vi "T2_Tau_Manipulation.vi"(8 "Numeric 2":i32, 9 "Invert?":bool, 10 "Numeric":i32, 11 "MW Step Size":dbl=2e-09) -> (3 "Tau":dbl)   [LabVIEW 2024]
uses:
  <vilib>/Utility/error.llb/DialogTypeEnum.ctl
  SpinCore_API_file_location.vi
panel:
  out "output array 2":T1(array[cluster])
  in  "clock_freq (MHz) 2":dbl=500.0
  out "x+y 11":dbl
  out "x+y 10":dbl
  out "x+y 9":dbl
  out "x+y 8":dbl
  out "x+y 7":dbl
  out "x+y 6":dbl
  out "x+y 5":dbl
  out "x+y 4":dbl
  out "x+y 3":dbl
  out "x+y 2":dbl
  out "output array":T1(array[cluster])
  in  "Instructions":T1(array[cluster])=[{"Instruct Data"=0, "Op Code"=0, "Flags"=[FALSE, FALSE, TRUE, FALSE, FALSE, FALSE, FALSE, TRUE, FALSE, FALSE, FALSE, FALSE, FALSE, FALSE, FALSE, FALSE, FALSE, FALSE, FALSE, FALSE, FALSE, FALSE, FALSE, TRUE], "Comments"="0 Triggers", "Time (s)"=1e-07}, {"Instruct Data"=0, "Op Code"=0, "Flags"=[FALSE, FALSE, FALSE, FALSE, FALSE, FALSE, FALSE, TRUE, FALSE, FALSE, FALSE, FALSE, FALSE, FALSE, FALSE, FALSE, FALSE, FALSE, FALSE, FALSE, FALSE, FALSE, FALSE, FALSE], "Comments"="1 Dark ", "Time (s)"=0.00017}, {"Instruct Data"=0, "Op Code"=0, "Flags"=[FALSE, FALSE, FALSE, FALSE, FALSE, FALSE, FALSE, TRUE, FALSE, FALSE, FALSE, FALSE, FALSE, FALSE, FALSE, FALSE, FALSE, FALSE, FALSE, FALSE, FALSE, FALSE, FALSE, FALSE], "Comments"="2 AOM Buffer", "Time (s)"=5e-07}, {"Instruct Data"=0, "Op Code"=0, "Flags"=[TRUE, FALSE, FALSE, TRUE, FALSE, FALSE, FALSE, TRUE, FALSE, FALSE, FALSE, FALSE, FALSE, FALSE, FALSE, FALSE, FALSE, FALSE, FALSE, FALSE, FALSE, FALSE, FALSE, FALSE], "Comments"="3 pi/2", "Time (s)"=3.7e-08}, {"Instruct Data"=0, "Op Code"=0, "Flags"=[FALSE, FALSE, FALSE, FALSE, FALSE, FALSE, FALSE, TRUE, FALSE, FALSE, FALSE, FALSE, FALSE, FALSE, FALSE, FALSE, FALSE, FALSE, FALSE, FALSE, FALSE, FALSE, FALSE, FALSE], "Comments"="4 tau", "Time (s)"=1e-08}, {"Instruct Data"=0, "Op Code"=0, "Flags"=[TRUE, FALSE, FALSE, TRUE, FALSE, FALSE, FALSE, TRUE, FALSE, FALSE, FALSE, FALSE, FALSE, FALSE, FALSE, FALSE, FALSE, FALSE, FALSE, FALSE, FALSE, FALSE, FALSE, FALSE], "Comments"="5  Pi_X", "Time (s)"=6.7e-08}, {"Instruct Data"=0, "Op Code"=0, "Flags"=[FALSE, FALSE, FALSE, FALSE, FALSE, FALSE, FALSE, TRUE, FALSE, FALSE, FALSE, FALSE, FALSE, FALSE, FALSE, FALSE, FALSE, FALSE, FALSE, FALSE, FALSE, FALSE, FALSE, FALSE], "Comments"="6 Tau", "Time (s)"=1e-08}, {"Instruct Data"=0, "Op Code"=0, "Flags"=[TRUE, FALSE, FALSE, TRUE, FALSE, FALSE, FALSE, TRUE, FALSE, FALSE, FALSE, FALSE, FALSE, FALSE, FALSE, FALSE, FALSE, FALSE, FALSE, FALSE, FALSE, FALSE, FALSE, FALSE], "Comments"="7 Pi/2", "Time (s)"=3.7e-08}, {"Instruct Data"=0, "Op Code"=0, "Flags"=[FALSE, TRUE, FALSE, FALSE, FALSE, FALSE, FALSE, TRUE, FALSE, FALSE, FALSE, FALSE, FALSE, FALSE, FALSE, FALSE, FALSE, FALSE, FALSE, FALSE, FALSE, FALSE, FALSE, FALSE], "Comments"="8 AOM", "Time (s)"=5e-07}, {"Instruct Data"=0, "Op Code"=0, "Flags"=[FALSE, TRUE, FALSE, FALSE, FALSE, FALSE, FALSE, FALSE, FALSE, FALSE, FALSE, FALSE, FALSE, FALSE, FALSE, FALSE, FALSE, FALSE, FALSE, FALSE, FALSE, FALSE, FALSE, FALSE], "Comments"="9 AOM non inhibit window", "Time (s)"=5e-07}, {"Instruct Data"=0, "Op Code"=0, "Flags"=[FALSE, TRUE, FALSE, FALSE, FALSE, FALSE, FALSE, TRUE, FALSE, FALSE, FALSE, FALSE, FALSE, FALSE, FALSE, FALSE, FALSE, FALSE, FALSE, FALSE, FALSE, FALSE, FALSE, FALSE], "Comments"="10 AOM Repolarization", "Time (s)"=4e-06}, {"Instruct Data"=0, "Op Code"=0, "Flags"=[FALSE, FALSE, FALSE, FALSE, FALSE, FALSE, FALSE, TRUE, FALSE, FALSE, FALSE, FALSE, FALSE, FALSE, FALSE, FALSE, FALSE, FALSE, FALSE, FALSE, FALSE, FALSE, FALSE, FALSE], "Comments"="11 Dark", "Time (s)"=0.00017}, {"Instruct Data"=0, "Op Code"=0, "Flags"=[FALSE, FALSE, FALSE, FALSE, FALSE, FALSE, FALSE, TRUE, FALSE, FALSE, FALSE, FALSE, FALSE, FALSE, FALSE, FALSE, FALSE, FALSE, FALSE, FALSE, FALSE, FALSE, FALSE, FALSE], "Comments"="12 AOM Buffer", "Time (s)"=5e-07}, {"Instruct Data"=0, "Op Code"=0, "Flags"=[TRUE, FALSE, FALSE, TRUE, FALSE, FALSE, FALSE, TRUE, FALSE, FALSE, FALSE, FALSE, FALSE, FALSE, FALSE, FALSE, FALSE, FALSE, FALSE, FALSE, FALSE, FALSE, FALSE, FALSE], "Comments"="13 Pi/2", "Time (s)"=3.7e-08}, {"Instruct Data"=0, "Op Code"=0, "Flags"=[FALSE, FALSE, FALSE, FALSE, FALSE, FALSE, FALSE, TRUE, FALSE, FALSE, FALSE, FALSE, FALSE, FALSE, FALSE, FALSE, FALSE, FALSE, FALSE, FALSE, FALSE, FALSE, FALSE, FALSE], "Comments"="14 tau", "Time (s)"=1e-08}, {"Instruct Data"=0, "Op Code"=0, "Flags"=[TRUE, FALSE, FALSE, FALSE, TRUE, FALSE, FALSE, TRUE, FALSE, FALSE, FALSE, FALSE, FALSE, FALSE, FALSE, FALSE, FALSE, FALSE, FALSE, FALSE, FALSE, FALSE, FALSE, FALSE], "Comments"="15 Pi_Y", "Time (s)"=6.9e-08}, {"Instruct Data"=0, "Op Code"=0, "Flags"=[FALSE, FALSE, FALSE, FALSE, FALSE, FALSE, FALSE, TRUE, FALSE, FALSE, FALSE, FALSE, FALSE, FALSE, FALSE, FALSE, FALSE, FALSE, FALSE, FALSE, FALSE, FALSE, FALSE, FALSE], "Comments"="16 tau", "Time (s)"=1e-08}, {"Instruct Data"=0, "Op Code"=0, "Flags"=[TRUE, FALSE, FALSE, TRUE, FALSE, FALSE, FALSE, TRUE, FALSE, FALSE, FALSE, FALSE, FALSE, FALSE, FALSE, FALSE, FALSE, FALSE, FALSE, FALSE, FALSE, FALSE, FALSE, FALSE], "Comments"="17 pi/2", "Time (s)"=3.7e-08}, {"Instruct Data"=0, "Op Code"=0, "Flags"=[FALSE, TRUE, FALSE, FALSE, FALSE, FALSE, FALSE, TRUE, FALSE, FALSE, FALSE, FALSE, FALSE, FALSE, FALSE, FALSE, FALSE, FALSE, FALSE, FALSE, FALSE, FALSE, FALSE, FALSE], "Comments"="18 AOM Delay", "Time (s)"=5e-07}, {"Instruct Data"=0, "Op Code"=0, "Flags"=[FALSE, TRUE, FALSE, FALSE, FALSE, FALSE, FALSE, FALSE, FALSE, FALSE, FALSE, FALSE, FALSE, FALSE, FALSE, FALSE, FALSE, FALSE, FALSE, FALSE, FALSE, FALSE, FALSE, FALSE], "Comments"="19 AOM non inhibit window", "Time (s)"=5e-07}, {"Instruct Data"=0, "Op Code"=6, "Flags"=[FALSE, TRUE, FALSE, FALSE, FALSE, FALSE, FALSE, TRUE, FALSE, FALSE, FALSE, FALSE, FALSE, FALSE, FALSE, FALSE, FALSE, FALSE, FALSE, FALSE, FALSE, FALSE, FALSE, FALSE], "Comments"="20  AOM Repolarization", "Time (s)"=4e-06}] {"Time (s)" format="%.3p"; "Op Code" items=["Continue", "Stop", "Loop", "End Loop", "JSR", "RTS", "Branch", "Long Delay", "Wait"]}
  in  "# of Instructions":u32=21
  in  "clock_freq (MHz)":dbl=500.0
  # "1)MW indicator\n2)AOM\n3)SR400 trigger\n4) I\n5) Q\n8) Inhibit\n24) Scope Trigger"
  # "1"
  # "2"
  # "3"
  # "4"
  # "5"
  # "6"
  # "7"
  # "8"
  # "9"
  # "10"
  # "11"
  # "12"
  # "13"
  # "14"
  # "15"
  # "16"
  # "17"
  # "18"
  # "19"
  # "20"
  # "21"
  # "22"
  # "23"
  # "24"
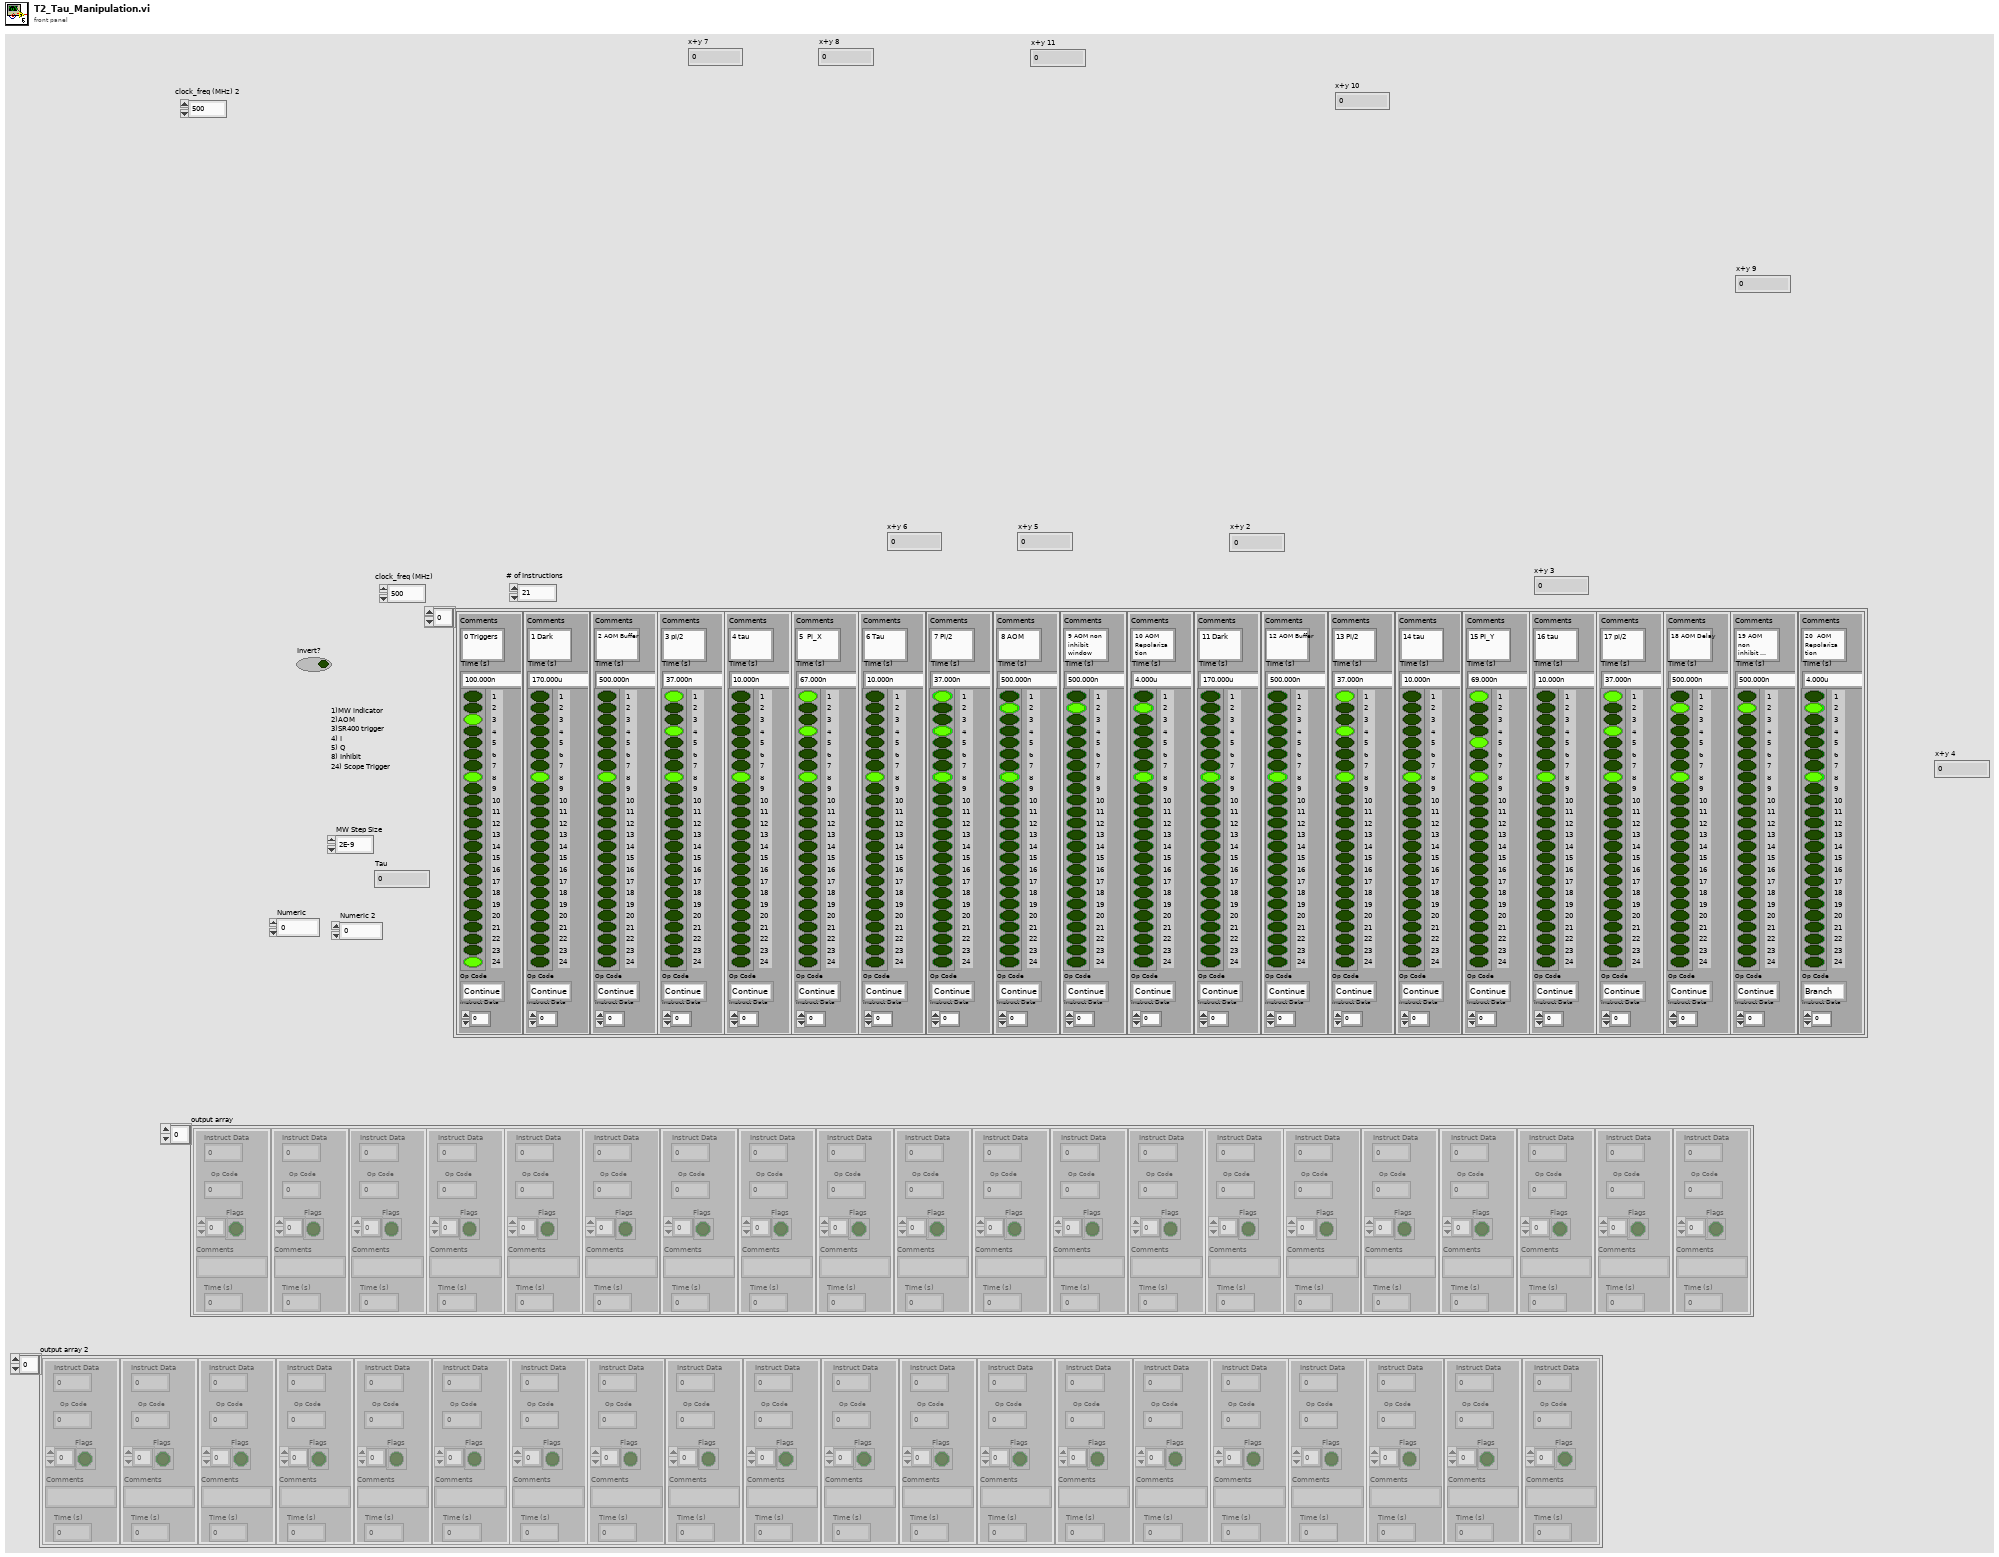
[diagram p1: front panel]
types:
  T1 = cluster{"Instruct Data":i32, "Op Code":i32, "Flags":bool[], "Comments":string, "Time (s)":dbl}[]
  T2 = typedef "DialogTypeEnum.ctl" = enum16{"no dialog", "OK message", "continue or stop message", "auto error handling dialog", "OK message + warnings", "continue/stop + warnings"}
  T3 = enum16{"Pulse Program", "Frequency Registers", "TX Phase Registers", "RX Phase Registers"}
  T4 = cluster{"Instruct Data":i32, "Op Code":i32, "Flags":bool[], "Comments":string, "Time (s)":dbl}
  T5 = cluster{"Instruct Data":i32, "Op Code":i32, "Flags":bool[], "Comments":string, dbl}
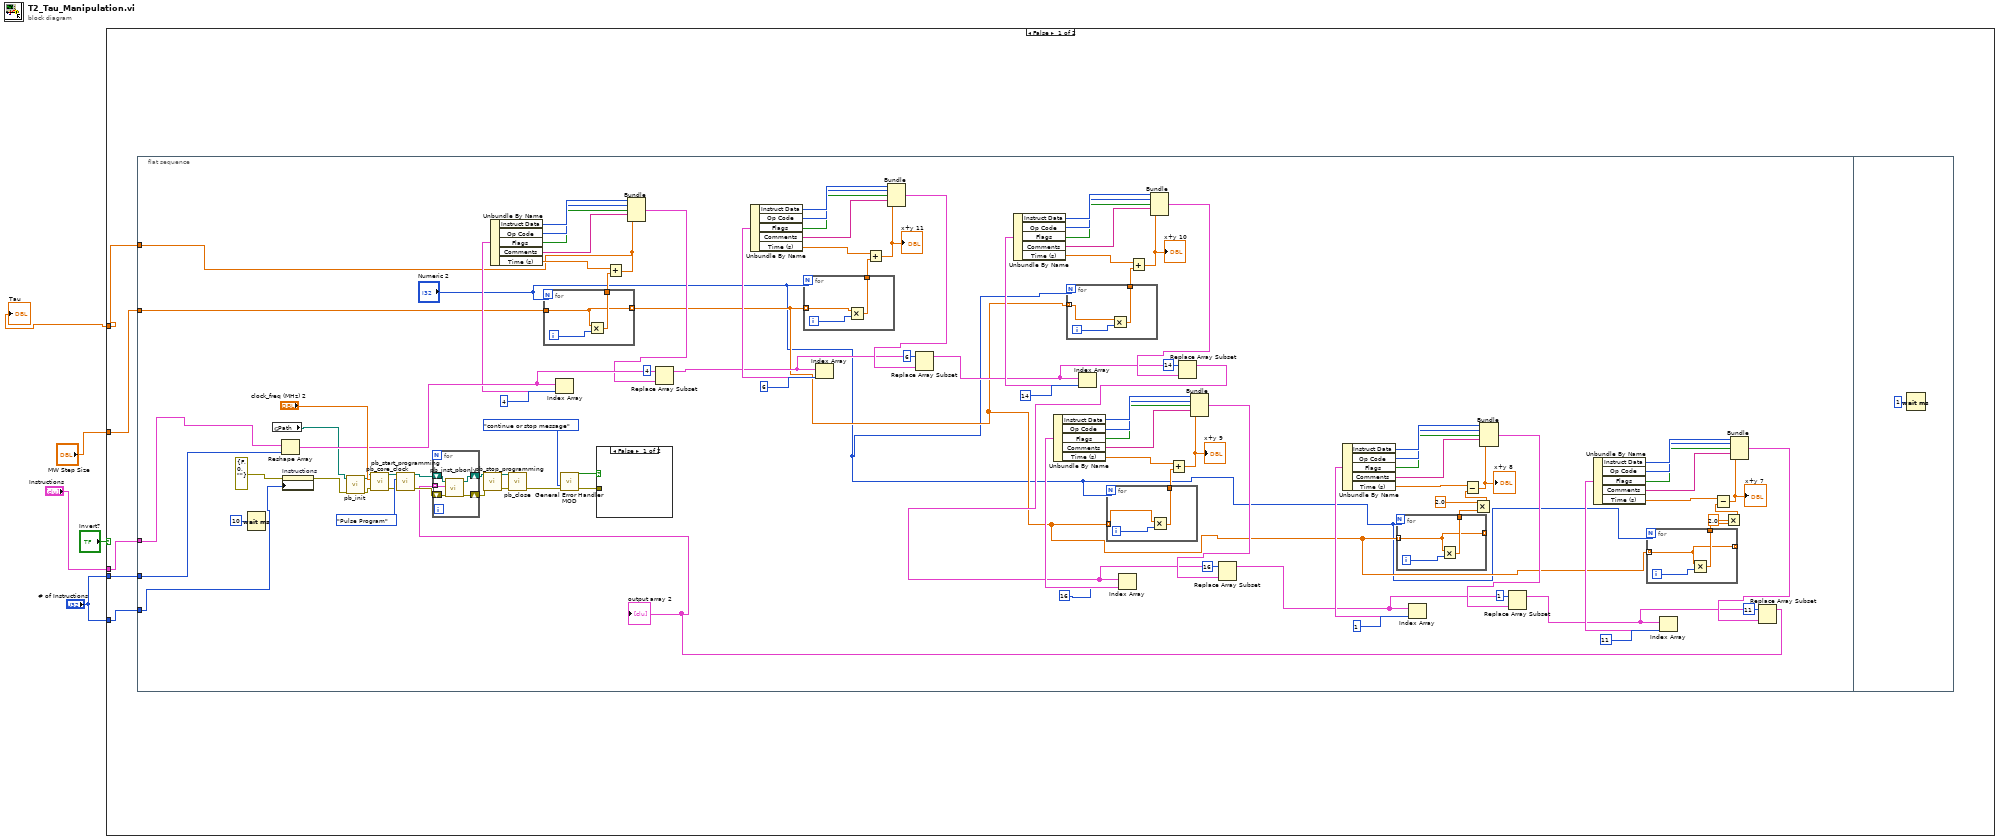
[diagram p0: block diagram]
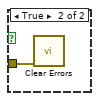
[diagram p2: hidden frame]
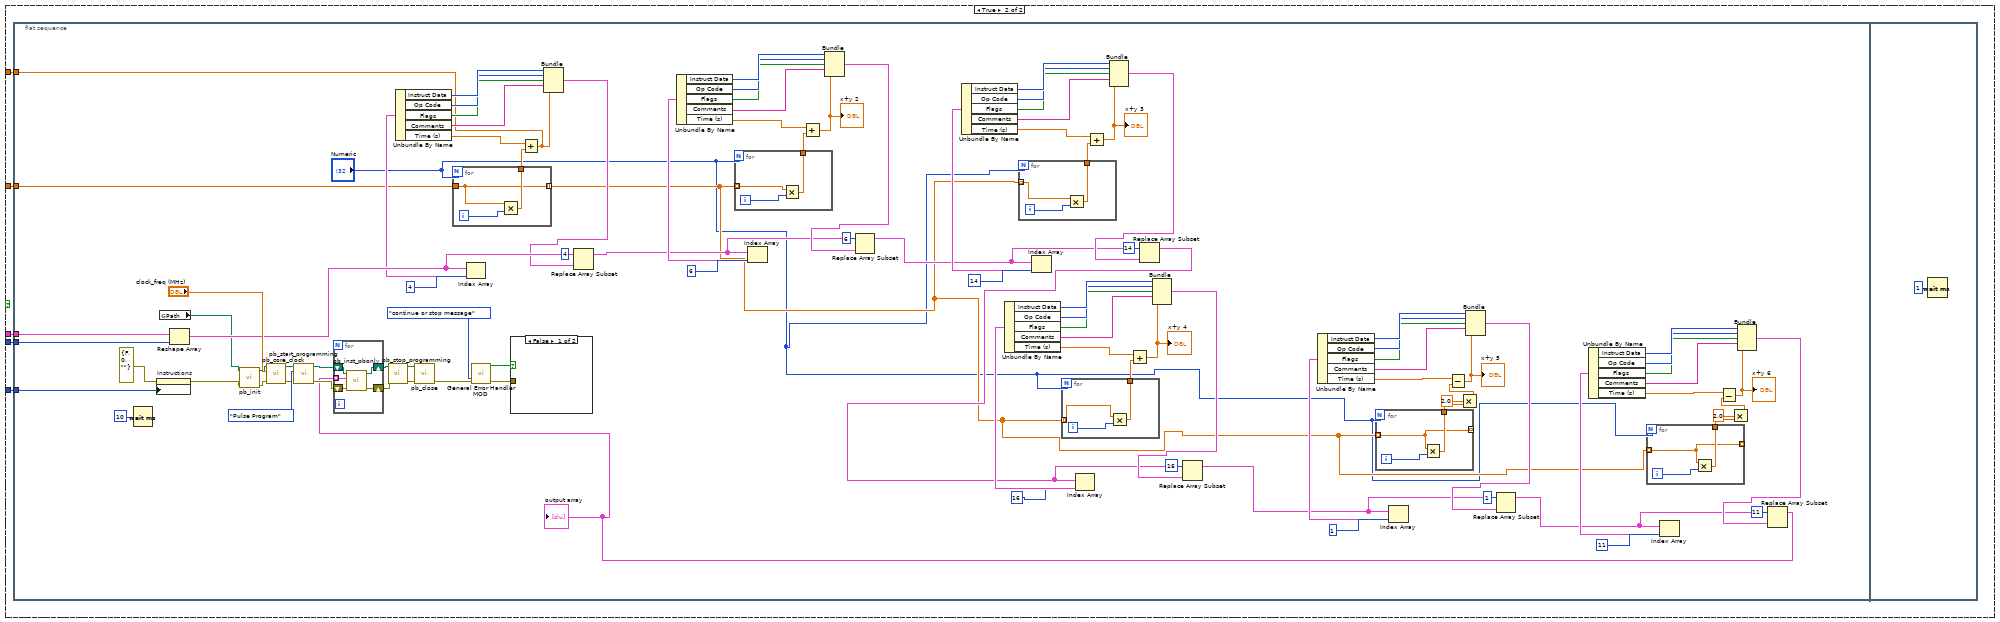
[diagram p3: hidden frame]
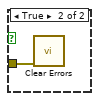
[diagram p4: hidden frame]
diagram:
  n1 = case shown="False" "Invert?" {
    tunnel: "Instructions" -> [w10 w143]
    tunnel: "# of Instructions" -> [w9 w142]
    tunnel: "# of Instructions" -> [w8 w141]
    tunnel: "MW Step Size" -> [w7 w140]
    tunnel: [w6 w139] -> w1
    frame False {
      n2 = flat-sequence {
        tunnel: w10 -> [w19]
        tunnel: w9 -> [w18]
        tunnel: w8 -> [w17]
        tunnel: w7 -> [w13]
        tunnel: [w12] -> w6
        frame #0 {
          n3 = Wait (ms)(milliseconds to wait=u32 10) -> ()  [unwired: 1 out]
          n4 = global read "SpinCore_API_file_location.vi" "Path"() -> (w14:path)
          n5 = Reshape Array "Reshape Array"(w19, w18) -> (w93:T1)
          n6 = property on="Instructions" class="Arr (strict)"(error in=errorcluster {"status"=FALSE, "code"=0, "source"=""} ("error in (no error)"), "Number of Columns"=w17) -> (error out=w15:errorcluster)  [unwired: 1 in, 1 out]
          n7 = call "pb_init.vi"("error in (no error)"=w15, "path in"=w14) -> ("error out"=w88:errorcluster, "path out"=w87:path)  [unwired: 8 in]
          n8 = call "pb_core_clock.vi"("error in (no error)"=w88, "clock_freq (MHz)"="clock_freq (MHz) 2", "path in"=w87) -> ("error out"=w102:errorcluster, "path out"=w103:path)  [unwired: 7 in]
          n9 = call "pb_start_programming.vi"("error in (no error)"=w102, "Device"=T3."Pulse Program", "path in"=w103) -> ("error out"=w109:errorcluster, "path out"=w113:path)  [unwired: 1 in, 6 out]
          n10 = for {
            N: "Numeric 2" -> [_]
            tunnel: [w130] -> w89
            tunnel: [w129] -> w20 mode=indexing
            tunnel: w13 -> [w129]
            i -> [w131]
            n11 = Multiply(x=w129, y=w131) -> (x*y=w130:dbl)
          }
          n12 = Index Array "Index Array"(array=w93, index=4) -> (element=w92:T4)
          n13 = Unbundle By Name "Unbundle By Name"(w92) -> ("Instruct Data"=w98:i32, "Op Code"=w97:i32, "Flags"=w96:bool[], "Comments"=w95:string, "Time (s)"=w94:dbl)
          n14 = Add(x=w94, y=w89) -> (x+y=w12:dbl)
          n15 = Bundle("Instruct Data"=w98, "Op Code"=w97, "Flags"=w96, "Comments"=w95, w12) -> (w90:T5)  [unwired: 1 in]
          n16 = Replace Array Subset "Replace Array Subset"(array=w93, new element=w90, index=4) -> (w74:T1)
          n17 = for {
            N: "Numeric 2" -> [_]
            tunnel: [w127] -> w75
            tunnel: w20 -> [w126] mode=indexing
            i -> [w128]
            n18 = Multiply(x=w126, y=w128) -> (x*y=w127:dbl)
          }
          n19 = Index Array "Index Array"(array=w74, index=6) -> (element=w78:T4)
          n20 = Unbundle By Name "Unbundle By Name"(w78) -> ("Instruct Data"=w84:i32, "Op Code"=w83:i32, "Flags"=w82:bool[], "Comments"=w81:string, "Time (s)"=w80:dbl)
          n21 = Add(x=w80, y=w75) -> (x+y=w79:dbl)
          "x+y 11" <- w79
          n22 = Bundle("Instruct Data"=w84, "Op Code"=w83, "Flags"=w82, "Comments"=w81, w79) -> (w76:T5)  [unwired: 1 in]
          n23 = Replace Array Subset "Replace Array Subset"(array=w74, new element=w76, index=6) -> (w62:T1)
          n24 = for {
            N: "Numeric 2" -> [_]
            tunnel: [w124] -> w63
            tunnel: w20 -> [w123] mode=indexing
            i -> [w125]
            n25 = Multiply(x=w123, y=w125) -> (x*y=w124:dbl)
          }
          n26 = Index Array "Index Array"(array=w62, index=14) -> (element=w66:T4)
          n27 = Unbundle By Name "Unbundle By Name"(w66) -> ("Instruct Data"=w72:i32, "Op Code"=w71:i32, "Flags"=w70:bool[], "Comments"=w69:string, "Time (s)"=w68:dbl)
          n28 = for {
            N: "Numeric 2" -> [_]
            tunnel: [w121] -> w52
            tunnel: w20 -> [w120] mode=indexing
            i -> [w122]
            n29 = Multiply(x=w120, y=w122) -> (x*y=w121:dbl)
          }
          n30 = Add(x=w68, y=w63) -> (x+y=w67:dbl)
          "x+y 10" <- w67
          n31 = Bundle("Instruct Data"=w72, "Op Code"=w71, "Flags"=w70, "Comments"=w69, w67) -> (w64:T5)  [unwired: 1 in]
          n32 = Replace Array Subset "Replace Array Subset"(array=w62, new element=w64, index=14) -> (w51:T1)
          n33 = Index Array "Index Array"(array=w51, index=16) -> (element=w55:T4)
          n34 = Unbundle By Name "Unbundle By Name"(w55) -> ("Instruct Data"=w61:i32, "Op Code"=w60:i32, "Flags"=w59:bool[], "Comments"=w58:string, "Time (s)"=w57:dbl)
          n35 = Add(x=w57, y=w52) -> (x+y=w56:dbl)
          "x+y 9" <- w56
          n36 = Bundle("Instruct Data"=w61, "Op Code"=w60, "Flags"=w59, "Comments"=w58, w56) -> (w53:T5)  [unwired: 1 in]
          n37 = Replace Array Subset "Replace Array Subset"(array=w51, new element=w53, index=16) -> (w39:T1)
          n38 = for {
            N: "Numeric 2" -> [_]
            tunnel: [w118] -> w38
            tunnel: [w117] -> _ mode=indexing
            tunnel: w20 -> [w117] mode=indexing
            i -> [w119]
            n39 = Multiply(x=w117, y=w119) -> (x*y=w118:dbl)
          }
          n40 = Index Array "Index Array"(array=w39, index=1) -> (element=w42:T4)
          n41 = Unbundle By Name "Unbundle By Name"(w42) -> ("Instruct Data"=w48:i32, "Op Code"=w47:i32, "Flags"=w46:bool[], "Comments"=w45:string, "Time (s)"=w44:dbl)
          n42 = Multiply(x=2.0, y=w38) -> (x*y=w36:dbl)
          n43 = Subtract(x=w44, y=w36) -> (x-y=w43:dbl)
          "x+y 8" <- w43
          n44 = Bundle("Instruct Data"=w48, "Op Code"=w47, "Flags"=w46, "Comments"=w45, w43) -> (w40:T5)  [unwired: 1 in]
          n45 = Replace Array Subset "Replace Array Subset"(array=w39, new element=w40, index=1) -> (w22:T1)
          n46 = for {
            N: "Numeric 2" -> [_]
            tunnel: [w115] -> w25
            tunnel: [w114] -> _ mode=indexing
            tunnel: w20 -> [w114] mode=indexing
            i -> [w116]
            n47 = Multiply(x=w114, y=w116) -> (x*y=w115:dbl)
          }
          n48 = Index Array "Index Array"(array=w22, index=11) -> (element=w28:T4)
          n49 = Unbundle By Name "Unbundle By Name"(w28) -> ("Instruct Data"=w34:i32, "Op Code"=w33:i32, "Flags"=w32:bool[], "Comments"=w31:string, "Time (s)"=w30:dbl)
          n50 = Multiply(x=2.0, y=w25) -> (x*y=w23:dbl)
          n51 = Subtract(x=w30, y=w23) -> (x-y=w29:dbl)
          "x+y 7" <- w29
          n52 = Bundle("Instruct Data"=w34, "Op Code"=w33, "Flags"=w32, "Comments"=w31, w29) -> (w26:T5)  [unwired: 1 in]
          n53 = Replace Array Subset "Replace Array Subset"(array=w22, new element=w26, index=11) -> (w21:T1)
          "output array 2" <- w21
          n54 = for {
            tunnel: w21 -> [w134] mode=indexing
            shift-right: [w136] -> w111
            shift-left: w113 -> [w137]
            shift-right: [w133] -> w108
            shift-left: w109 -> [w135]
            n55 = call "pb_inst_pbonly.vi"("error in (no error)"=w135, "PB Instruction"=w134, "path in"=w137) -> ("error out"=w133:errorcluster, "path out"=w136:path)  [unwired: 2 in, 5 out]
          }
          n56 = call "pb_stop_programming.vi"("error in (no error)"=w108, "path in"=w111) -> ("error out"=w107:errorcluster, "path out"=w112:path)  [unwired: 1 in, 7 out]
          n57 = call "pb_close.vi"("error in (no error)"=w107, "path in"=w112) -> ("error out"=w100:errorcluster)  [unwired: 9 out]
          n58 = call "General Error Handler MOD.vi"("type of dialog (OK msg:1)"=DialogTypeEnum."continue or stop message", "error in (no error)"=w100) -> ("STOP?"=w104:bool, "error out"=w105:errorcluster)  [unwired: 12 out]
          n59 = case shown="False" w104 {
            tunnel: w105 -> [_ w132]
            frame False {
            }
            frame True {
              n60 = call <vilib>:"Clear Errors.vi"("error in (no error)"=w132) -> ()  [unwired: 1 in, 6 out]
            }
          }
        }
        frame #1 {
          n61 = Wait (ms)(milliseconds to wait=u32 1) -> ()  [unwired: 1 out]
        }
      }
    }
    frame True {
      n62 = flat-sequence {
        tunnel: w143 -> [w149]
        tunnel: w142 -> [w148]
        tunnel: w141 -> [w147]
        tunnel: w140 -> [w146]
        tunnel: [w145] -> w139
        frame #0 {
          n63 = Wait (ms)(milliseconds to wait=u32 10) -> ()  [unwired: 1 out]
          n64 = property on="Instructions" class="Arr (strict)"(error in=errorcluster {"status"=FALSE, "code"=0, "source"=""} ("error in (no error)"), "Number of Columns"=w147) -> (error out=w220:errorcluster)  [unwired: 1 in, 1 out]
          n65 = global read "SpinCore_API_file_location.vi" "Path"() -> (w221:path)
          n66 = Reshape Array "Reshape Array"(w149, w148) -> (w226:T1)
          n67 = call "pb_init.vi"("error in (no error)"=w220, "path in"=w221) -> ("error out"=w219:errorcluster, "path out"=w218:path)  [unwired: 8 in]
          n68 = call "pb_core_clock.vi"("error in (no error)"=w219, "clock_freq (MHz)"="clock_freq (MHz)", "path in"=w218) -> ("error out"=w235:errorcluster, "path out"=w236:path)  [unwired: 7 in]
          n69 = call "pb_start_programming.vi"("error in (no error)"=w235, "Device"=T3."Pulse Program", "path in"=w236) -> ("error out"=w242:errorcluster, "path out"=w246:path)  [unwired: 1 in, 6 out]
          n70 = for {
            N: "Numeric" -> [_]
            tunnel: [w263] -> w222
            tunnel: [w262] -> w150 mode=indexing
            tunnel: w146 -> [w262]
            i -> [w264]
            n71 = Multiply(x=w262, y=w264) -> (x*y=w263:dbl)
          }
          n72 = Index Array "Index Array"(array=w226, index=4) -> (element=w225:T4)
          n73 = Unbundle By Name "Unbundle By Name"(w225) -> ("Instruct Data"=w231:i32, "Op Code"=w230:i32, "Flags"=w229:bool[], "Comments"=w228:string, "Time (s)"=w227:dbl)
          n74 = Add(x=w227, y=w222) -> (x+y=w145:dbl)
          n75 = Bundle("Instruct Data"=w231, "Op Code"=w230, "Flags"=w229, "Comments"=w228, w145) -> (w223:T5)  [unwired: 1 in]
          n76 = Replace Array Subset "Replace Array Subset"(array=w226, new element=w223, index=4) -> (w204:T1)
          n77 = for {
            N: "Numeric" -> [_]
            tunnel: [w260] -> w205
            tunnel: w150 -> [w259] mode=indexing
            i -> [w261]
            n78 = Multiply(x=w259, y=w261) -> (x*y=w260:dbl)
          }
          n79 = Index Array "Index Array"(array=w204, index=6) -> (element=w208:T4)
          n80 = Unbundle By Name "Unbundle By Name"(w208) -> ("Instruct Data"=w214:i32, "Op Code"=w213:i32, "Flags"=w212:bool[], "Comments"=w211:string, "Time (s)"=w210:dbl)
          n81 = Add(x=w210, y=w205) -> (x+y=w209:dbl)
          "x+y 2" <- w209
          n82 = Bundle("Instruct Data"=w214, "Op Code"=w213, "Flags"=w212, "Comments"=w211, w209) -> (w206:T5)  [unwired: 1 in]
          n83 = Replace Array Subset "Replace Array Subset"(array=w204, new element=w206, index=6) -> (w192:T1)
          n84 = for {
            N: "Numeric" -> [_]
            tunnel: [w257] -> w193
            tunnel: w150 -> [w256] mode=indexing
            i -> [w258]
            n85 = Multiply(x=w256, y=w258) -> (x*y=w257:dbl)
          }
          n86 = Index Array "Index Array"(array=w192, index=14) -> (element=w196:T4)
          n87 = Unbundle By Name "Unbundle By Name"(w196) -> ("Instruct Data"=w202:i32, "Op Code"=w201:i32, "Flags"=w200:bool[], "Comments"=w199:string, "Time (s)"=w198:dbl)
          n88 = for {
            N: "Numeric" -> [_]
            tunnel: [w254] -> w182
            tunnel: w150 -> [w253] mode=indexing
            i -> [w255]
            n89 = Multiply(x=w253, y=w255) -> (x*y=w254:dbl)
          }
          n90 = Add(x=w198, y=w193) -> (x+y=w197:dbl)
          "x+y 3" <- w197
          n91 = Bundle("Instruct Data"=w202, "Op Code"=w201, "Flags"=w200, "Comments"=w199, w197) -> (w194:T5)  [unwired: 1 in]
          n92 = Replace Array Subset "Replace Array Subset"(array=w192, new element=w194, index=14) -> (w181:T1)
          n93 = Index Array "Index Array"(array=w181, index=16) -> (element=w185:T4)
          n94 = Unbundle By Name "Unbundle By Name"(w185) -> ("Instruct Data"=w191:i32, "Op Code"=w190:i32, "Flags"=w189:bool[], "Comments"=w188:string, "Time (s)"=w187:dbl)
          n95 = Add(x=w187, y=w182) -> (x+y=w186:dbl)
          "x+y 4" <- w186
          n96 = Bundle("Instruct Data"=w191, "Op Code"=w190, "Flags"=w189, "Comments"=w188, w186) -> (w183:T5)  [unwired: 1 in]
          n97 = Replace Array Subset "Replace Array Subset"(array=w181, new element=w183, index=16) -> (w169:T1)
          n98 = for {
            N: "Numeric" -> [_]
            tunnel: [w251] -> w168
            tunnel: [w250] -> _ mode=indexing
            tunnel: w150 -> [w250] mode=indexing
            i -> [w252]
            n99 = Multiply(x=w250, y=w252) -> (x*y=w251:dbl)
          }
          n100 = Index Array "Index Array"(array=w169, index=1) -> (element=w172:T4)
          n101 = Unbundle By Name "Unbundle By Name"(w172) -> ("Instruct Data"=w178:i32, "Op Code"=w177:i32, "Flags"=w176:bool[], "Comments"=w175:string, "Time (s)"=w174:dbl)
          n102 = Multiply(x=2.0, y=w168) -> (x*y=w166:dbl)
          n103 = Subtract(x=w174, y=w166) -> (x-y=w173:dbl)
          "x+y 5" <- w173
          n104 = Bundle("Instruct Data"=w178, "Op Code"=w177, "Flags"=w176, "Comments"=w175, w173) -> (w170:T5)  [unwired: 1 in]
          n105 = Replace Array Subset "Replace Array Subset"(array=w169, new element=w170, index=1) -> (w152:T1)
          n106 = for {
            N: "Numeric" -> [_]
            tunnel: [w248] -> w155
            tunnel: [w247] -> _ mode=indexing
            tunnel: w150 -> [w247] mode=indexing
            i -> [w249]
            n107 = Multiply(x=w247, y=w249) -> (x*y=w248:dbl)
          }
          n108 = Index Array "Index Array"(array=w152, index=11) -> (element=w158:T4)
          n109 = Unbundle By Name "Unbundle By Name"(w158) -> ("Instruct Data"=w164:i32, "Op Code"=w163:i32, "Flags"=w162:bool[], "Comments"=w161:string, "Time (s)"=w160:dbl)
          n110 = Multiply(x=2.0, y=w155) -> (x*y=w153:dbl)
          n111 = Subtract(x=w160, y=w153) -> (x-y=w159:dbl)
          "x+y 6" <- w159
          n112 = Bundle("Instruct Data"=w164, "Op Code"=w163, "Flags"=w162, "Comments"=w161, w159) -> (w156:T5)  [unwired: 1 in]
          n113 = Replace Array Subset "Replace Array Subset"(array=w152, new element=w156, index=11) -> (w151:T1)
          "output array" <- w151
          n114 = for {
            tunnel: w151 -> [w267] mode=indexing
            shift-right: [w269] -> w244
            shift-left: w246 -> [w270]
            shift-right: [w266] -> w241
            shift-left: w242 -> [w268]
            n115 = call "pb_inst_pbonly.vi"("error in (no error)"=w268, "PB Instruction"=w267, "path in"=w270) -> ("error out"=w266:errorcluster, "path out"=w269:path)  [unwired: 2 in, 5 out]
          }
          n116 = call "pb_stop_programming.vi"("error in (no error)"=w241, "path in"=w244) -> ("error out"=w240:errorcluster, "path out"=w245:path)  [unwired: 1 in, 7 out]
          n117 = call "pb_close.vi"("error in (no error)"=w240, "path in"=w245) -> ("error out"=w233:errorcluster)  [unwired: 9 out]
          n118 = call "General Error Handler MOD.vi"("type of dialog (OK msg:1)"=DialogTypeEnum."continue or stop message", "error in (no error)"=w233) -> ("STOP?"=w237:bool, "error out"=w238:errorcluster)  [unwired: 12 out]
          n119 = case shown="False" w237 {
            tunnel: w238 -> [_ w265]
            frame False {
            }
            frame True {
              n120 = call <vilib>:"Clear Errors.vi"("error in (no error)"=w265) -> ()  [unwired: 1 in, 6 out]
            }
          }
        }
        frame #1 {
          n121 = Wait (ms)(milliseconds to wait=u32 1) -> ()  [unwired: 1 out]
        }
      }
    }
  }
  "Tau" <- w1
